vi "2_WF_Anomaly_Detection(Threshold_Evaluation).vi"() -> ()   [LabVIEW 2020]
uses:
  Controls/Optimal_Threshold_Range'.ctl
  <vilib>/Ngene/Deep Learning Toolkit/Toolkit/NN_Network/Controls/NN_Save_Before_Destroy_Options.ctl
  <vilib>/Ngene/Deep Learning Toolkit/Toolkit/NN_Data/subVIs/Get_Data_Vals/2D/NN_Data_Get_ValByRef(2D_SGL).vi
  <vilib>/Ngene/Deep Learning Toolkit/Toolkit/NN_Network/subVIs/NN_Predict/NN_Predict(In1D_Out1D).vi
  <vilib>/Ngene/Deep Learning Toolkit/Toolkit/NN_Data/subVIs/Dataset/NN_Variant_to_DVR/2D/NN_Data_Variant_to_DVR(2D_SGL).vi
  <vilib>/Ngene/Deep Learning Toolkit/Toolkit/Deep_Learning_Toolkit_by_Ngene.lvlib
  <vilib>/Analysis/NI_AALPro.lvlib
panel:
  in  "Validation (Abnormal Samples) dataset path":path=path "D:/working/Anomaly Detection/Validation/Abnormal"
  in  "Validation (Normal Samples) dataset path":path=path "D:/working/Anomaly Detection/Validation/Normal"
  out "Integrals of Normalized Anomaly Score Distributions":cluster{"Axis":dbl[], "Integral X":dbl[]}[](graph)
  out "Anomaly Score Distributions":T1(graph)=[{"X Values"=array[700 elements], "Histogram: h(x)"=[0, 0, 0, 0, 0, 0, 0, 0, 0, 0, 0, 0, 0, 0, 0, 0, 0, 0, 0, 0, 0, 0, 0, 0, 0, 0, 0, 0, 0, 0, 0, 0, 0, 1, 0, 0, 2, 2, 5, 2, 1, 11, 4, 7, 12, 11, 12, 12, 12, 16, 19, 10, 17, 15, 12, 14, 24, 15, 17, 16, 14, 7, 13, 13, 14, 6, 12, 16, 6, 11, 14, 2, 6, 4, 7, 7, 5, 6, 7, 7, 4, 4, 2, 8, 4, 2, 3, 1, 4, 0, 1, 1, 1, 5, 1, 3, 0, 1, 2, 0, 1, 1, 1, 1, 0, 0, 0, 0, 0, 0, 0, 0, 0, 2, 1, 0, 0, 0, 0, 0, 0, 0, 0, 0, 0, 0, 0, 0, 0, 0, 0, 0, 0, 0, 0, 0, 0, 0, 0, 0, 0, 0, 0, 0, 0, 0, 0, 0, 0, 0, 0, 0, 0, 0, 0, 0, 0, 0, 0, 0, 0, 0, 0, 0, 0, 0, 0, 0, 0, 0, 0, 0, 0, 0, 0, 0, 0, 0, 0, 0, 0, 0, 0, 0, 0, 0, 0, 0, 0, 0, 0, 0, 0, 0, 0, 0, 0, 0, 0, 0, 0, 0, 0, 0, 0, 0, 0, 0, 0, 0, 0, 0, 0, 0, 0, 0, 0, 0, 0, 0, 0, 0, 0, 0, 0, 0, 0, 0, 0, 0, 0, 0, 0, 0, 0, 0, 0, 0, 0, 0, 0, 0, 0, 0, 0, 0, 0, 0, 0, 0, 0, 0, 0, 0, 0, 0, 0, 0, 0, 0, 0, 0, 0, 0, 0, 0, 0, 0, 0, 0, 0, 0, 0, 0, 0, 0, 0, 0, 0, 0, 0, 0, 0, 0, 0, 0, 0, 0, 0, 0, 0, 0, 0, 0, 0, 0, 0, 0, 0, 0, 0, 0, 0, 0, 0, 0, 0, 0, 0, 0, 0, 0, 0, 0, 0, 0, 0, 0, 0, 0, 0, 0, 0, 0, 0, 0, 0, 0, 0, 0, 0, 0, 0, 0, 0, 0, 0, 0, 0, 0, 0, 0, 0, 0, 0, 0, 0, 0, 0, 0, 0, 0, 0, 0, 0, 0, 0, 0, 0, 0, 0, 0, 0, 0, 0, 0, 0, 0, 0, 0, 0, 0, 0, 0, 0, 0, 0, 0, 0, 0, 0, 0, 0, 0, 0, 0, 0, 0, 0, 0, 0, 0, 0, 0, 0, 0, 0, 0, 0, 0, 0, 0, 0, 0, 0, 0, 0, 0, 0, 0, 0, 0, 0, 0, 0, 0, 0, 0, 0, 0, 0, 0, 0, 0, 0, 0, 0, 0, 0, 0, 0, 0, 0, 0, 0, 0, 0, 0, 0, 0, 0, 0, 0, 0, 0, 0, 0, 0, 0, 0, 0, 0, 0, 0, 0, 0, 0, 0, 0, 0, 0, 0, 0, 0, 0, 0, 0, 0, 0, 0, 0, 0, 0, 0, 0, 0, 0, 0, 0, 0, 0, 0, 0, 0, 0, 0, 0, 0, 0, 0, 0, 0, 0, 0, 0, 0, 0, 0, 0, 0, 0, 0, 0, 0, 0, 0, 0, 0, 0, 0, 0, 0, 0, 0, 0, 0, 0, 0, 0, 0, 0, 0, 0, 0, 0, 0, 0, 0, 0, 0, 0, 0, 0, 0, 0, 0, 0, 0, 0, 0, 0, 0, 0, 0, 0, 0, 0, 0, 0, 0, 0, 0, 0, 0, 0, 0, 0, 0, 0, 0, 0, 0, 0, 0, 0, 0, 0, 0, 0, 0, 0, 0, 0, 0, 0, 0, 0, 0, 0, 0, 0, 0, 0, 0, 0, 0, 0, 0, 0, 0, 0, 0, 0, 0, 0, 0, 0, 0, 0, 0, 0, 0, 0, 0, 0, 0, 0, 0, 0, 0, 0, 0, 0, 0, 0, 0, 0, 0, 0, 0, 0, 0, 0, 0, 0, 0, 0, 0, 0, 0, 0, 0, 0, 0, 0, 0, 0, 0, 0, 0, 0, 0, 0, 0, 0, 0, 0, 0, 0, 0, 0, 0, 0, 0, 0, 0, 0, 0, 0, 0, 0, 0, 0, 0, 0, 0, 0, 0, 0, 0, 0, 0, 0, 0, 0, 0, 0, 0, 0, 0, 0, 0, 0, 0, 0, 0, 0, 0, 0, 0, 0, 0, 0, 0, 0, 0, 0, 0, 0, 0]}, {"X Values"=array[700 elements], "Histogram: h(x)"=[0, 0, 0, 0, 0, 0, 0, 0, 0, 0, 0, 0, 0, 0, 0, 0, 0, 0, 0, 0, 0, 0, 0, 0, 0, 0, 0, 0, 0, 0, 0, 0, 0, 0, 0, 0, 0, 0, 0, 0, 0, 0, 0, 0, 0, 0, 0, 0, 0, 0, 0, 0, 0, 0, 0, 0, 0, 0, 0, 0, 0, 0, 0, 0, 0, 0, 0, 0, 0, 0, 0, 0, 0, 0, 0, 0, 0, 0, 0, 0, 0, 0, 0, 0, 0, 0, 0, 0, 0, 0, 0, 0, 0, 0, 0, 0, 0, 0, 0, 0, 0, 0, 0, 0, 0, 0, 0, 0, 0, 0, 0, 0, 0, 0, 0, 0, 0, 0, 0, 0, 0, 0, 0, 0, 0, 0, 0, 0, 0, 0, 0, 0, 0, 0, 0, 0, 0, 0, 0, 0, 0, 0, 0, 0, 0, 0, 0, 0, 0, 0, 0, 0, 0, 0, 0, 0, 0, 0, 0, 0, 0, 0, 0, 0, 0, 0, 0, 0, 0, 0, 1, 0, 0, 0, 0, 0, 1, 0, 0, 0, 0, 0, 0, 1, 0, 0, 0, 0, 0, 1, 0, 2, 2, 0, 0, 1, 2, 0, 0, 1, 0, 1, 2, 1, 5, 1, 0, 2, 3, 0, 0, 0, 4, 3, 2, 1, 2, 1, 2, 6, 1, 0, 0, 5, 0, 0, 2, 4, 1, 6, 0, 0, 4, 2, 2, 3, 4, 3, 3, 2, 2, 4, 4, 1, 6, 0, 3, 1, 1, 1, 2, 1, 0, 3, 2, 3, 2, 1, 2, 3, 4, 3, 1, 1, 1, 4, 3, 3, 3, 1, 1, 1, 4, 0, 2, 0, 2, 4, 2, 1, 1, 1, 1, 1, 0, 1, 0, 1, 1, 1, 1, 0, 2, 4, 1, 0, 2, 0, 0, 0, 0, 1, 1, 2, 0, 1, 0, 1, 2, 0, 1, 1, 0, 2, 2, 1, 1, 0, 1, 1, 3, 0, 1, 0, 0, 1, 1, 0, 1, 5, 2, 0, 2, 1, 1, 2, 1, 0, 0, 0, 1, 0, 2, 1, 0, 0, 0, 0, 0, 1, 2, 0, 1, 0, 0, 1, 0, 1, 1, 0, 3, 0, 0, 0, 4, 0, 0, 1, 0, 0, 2, 1, 3, 1, 2, 1, 2, 3, 1, 3, 2, 1, 3, 0, 2, 2, 1, 1, 0, 1, 0, 1, 4, 1, 1, 0, 1, 1, 1, 0, 0, 3, 0, 0, 3, 1, 2, 3, 2, 1, 0, 1, 2, 1, 1, 2, 1, 1, 3, 3, 1, 1, 1, 2, 1, 3, 3, 4, 2, 1, 1, 1, 0, 2, 0, 0, 5, 0, 0, 0, 2, 1, 2, 1, 4, 0, 1, 2, 0, 1, 1, 1, 3, 2, 1, 2, 2, 1, 0, 1, 0, 1, 1, 3, 2, 0, 2, 0, 1, 1, 0, 1, 1, 1, 2, 1, 1, 0, 0, 0, 0, 0, 0, 0, 0, 0, 0, 0, 1, 0, 0, 0, 1, 0, 1, 0, 1, 0, 0, 0, 0, 0, 0, 1, 0, 0, 0, 0, 0, 0, 0, 0, 0, 0, 0, 0, 0, 0, 0, 0, 0, 0, 0, 0, 0, 0, 0, 0, 0, 1, 0, 0, 0, 0, 0, 0, 0, 0, 0, 0, 2, 0, 0, 0, 0, 0, 0, 0, 0, 0, 0, 0, 0, 0, 0, 0, 0, 0, 0, 1, 0, 1, 1, 0, 1, 1, 0, 0, 0, 1, 0, 0, 0, 1, 1, 0, 2, 0, 2, 1, 2, 2, 0, 1, 0, 0, 1, 1, 1, 1, 2, 2, 1, 1, 0, 0, 0, 0, 3, 2, 1, 3, 1, 1, 2, 0, 4, 1, 1, 1, 0, 0, 1, 2, 1, 0, 5, 2, 1, 3, 0, 2, 1, 3, 0, 3, 2, 2, 0, 1, 0, 1, 2, 1, 1, 2, 3, 1, 0, 2, 0, 0, 0, 0, 0, 0, 1, 0, 0, 0, 0, 0, 0, 1, 1, 0, 0, 1, 2, 0, 0, 0, 0, 0, 0, 0, 1, 0, 0, 0, 0, 0, 0, 0, 0, 0, 0, 0, 0, 0, 0, 0, 0, 0, 0, 0, 0, 0, 0, 0, 0, 0, 0, 0, 0, 0, 0, 0, 0, 0]}]
  out "Optimal Threshold Range":T2={"Start"=0.16499999999999998, "Stop"=0.24214285714285716} {"Stop" format="%#_3g"; "Start" format="%#_3g"}
  in  "Weights File Path":path=path "D:/Ngene/GitHub/deepltk_examples/2_Waveform_Processing/24_Waveform_Anomaly_Detection/working/Anomaly_Detection/Anomaly_Detection_weights_25_06_11__13_26_24.bin"
  in  "CFG file path":path=path "D:/Ngene/GitHub/deepltk_examples/2_Waveform_Processing/24_Waveform_Anomaly_Detection/working/Anomaly_Detection/Anomaly_Detection_net_cfg_25_06_11__13_26_24.cfg"
  # "Overview: This VI is designed to calculate the optimal anomaly threshold.\nRequirements: Deep Learning Toolkit for LabVIEW - https://www.ngene.co/deep-learning-toolkit-for-labview\nInstructions:\n1. Provide \"Network Configuration File Path\" and \"Weight File Path\" generated from \"1_WF_Anomaly_Detection(Training).vi\".\n2. Provide Validation (Normal Samples) and Validation (Abnormal Samples) dataset paths.\n3. Run the VI.\n4.Observe the Range of optimal threshold values.\n5. Choose a value from the range of optimal threshold calculated after the VI stops, and use it as a anomaly detetcion threshold in \"3_WF_Anomaly_Detection(Accuracy_Evaluation).vi\" \n6. Open \"3_WF_Anomaly_Detection(Accuracy_Evaluation).vi\"  to deploy the trained network for inference."
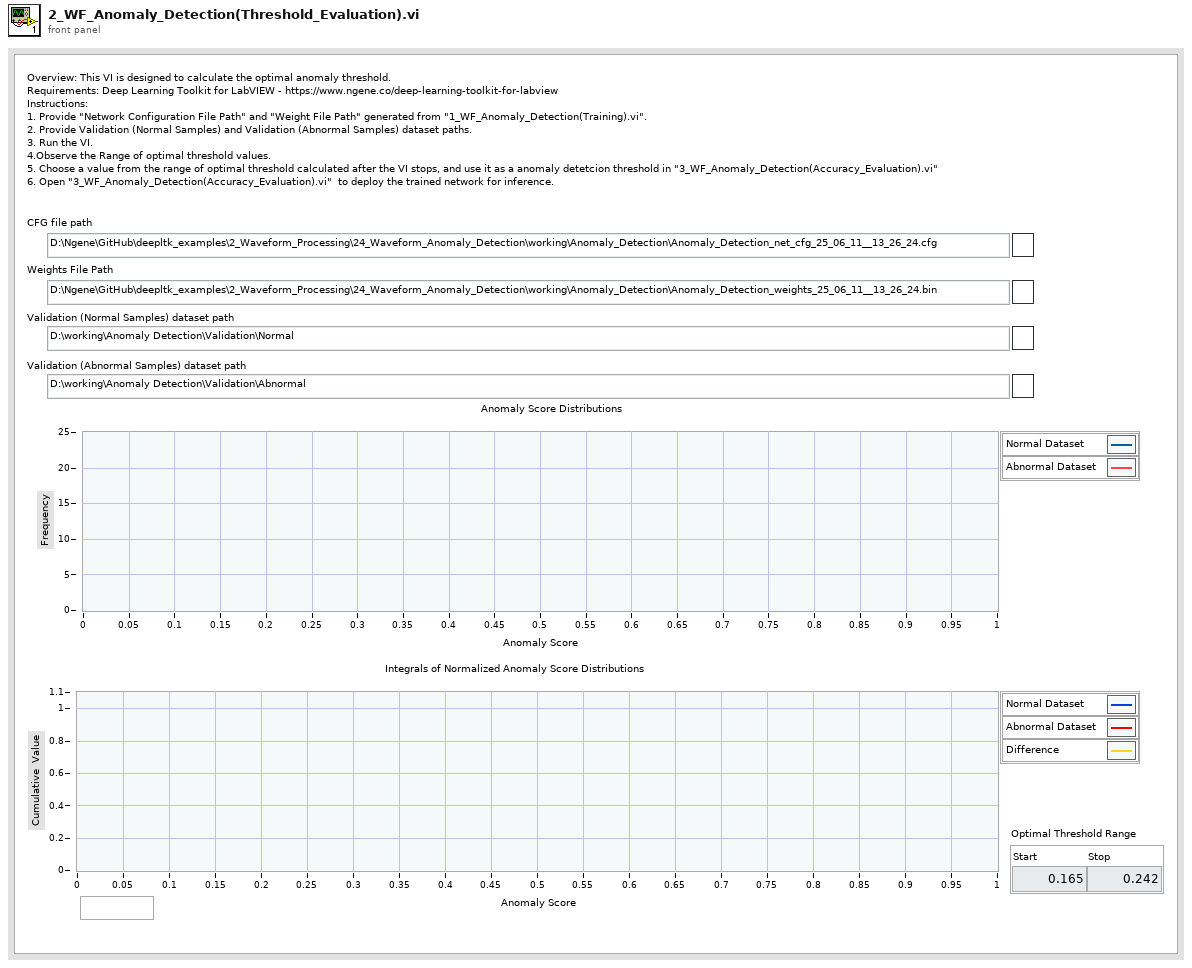
[diagram p1: front panel]
types:
  T1 = cluster{"X Values":dbl[], "Histogram: h(x)":i32[]}[]
  T2 = typedef "Optimal_Threshold_Range'.ctl" = cluster{"Start":dbl, "Stop":dbl}
  T3 = typedef "Deep_Learning_Toolkit_by_Ngene.lvlib/NN_Save_Before_Destroy_Options.ctl" = cluster{"CFG?":bool, "Weights?":bool, "Render?":bool}
  T4 = typedef "Deep_Learning_Toolkit_by_Ngene.lvlib/NN_Config_Params.ctl" = cluster{"Name":string, "mBatch":i32, "NN_Train_Params":T5, "LR_Decay_Policy":T8, "Labels":string[], "Loss":T10, "Max_WS_Size(B)":i64, "DryRun?":bool}
  T5 = typedef "Deep_Learning_Toolkit_by_Ngene.lvlib/NN_Train_Params.ctl" = cluster{"Optimizer":T6, "Beta_1":sgl, "Beta_2":sgl, "Weight Decay(L1)":sgl, "Weight Decay(L2)":sgl, "Data_Sampling":T7}
  T6 = typedef "Deep_Learning_Toolkit_by_Ngene.lvlib/NN_Train_Optimizer.ctl" = enum16{"SGD", "Adam", "Adagrad", "Adadelta", "RMSProp", "Nesterov"}
  T7 = typedef "Deep_Learning_Toolkit_by_Ngene.lvlib/NN_Train_Data_Sampling.ctl" = enum16{"Random", "Sequential"}
  T8 = typedef "Deep_Learning_Toolkit_by_Ngene.lvlib/NN_LR_Policy_Cfg.ctl" = cluster{"Policy_Type":T9, "LR0":dbl, "k":sgl, "WarmUp_Policy":enum16{"Step", "Ramp"}, "WarmUp_Iter":i32, "WarmUp_Ratio":sgl}
  T9 = typedef "Deep_Learning_Toolkit_by_Ngene.lvlib/NN_LR_Policy_Type.ctl" = enum16{"Manual", "Step", "Exp", "1/t"}
  T10 = typedef "Deep_Learning_Toolkit_by_Ngene.lvlib/NN_Loss_Config_Params.ctl" = cluster{"Loss_Type":T11, "Loss_Conf_Params":variant}
  T11 = typedef "Deep_Learning_Toolkit_by_Ngene.lvlib/NN_Loss_Type.ctl" = enum16{"None", "MSE", "CrossEntropy", "YOLO_v2", "YOLO_v4"}
  T12 = typedef "Deep_Learning_Toolkit_by_Ngene.lvlib/NN_Layer_Config_Params.ctl" = cluster{"Layer_Type":T13, "Layer_Conf_Params":variant, "Input Layers":string[]}
  T13 = typedef "Deep_Learning_Toolkit_by_Ngene.lvlib/NN_Layer_Type.ctl" = enum16{"Input1D", "Input3D", "Conv1D", "Conv2D", "Conv2D_Adv", "MaxPool", "AvgPool", "UpSample", "DropOut3D", "ShortCut", "Concat", "SoftMax3D", "FC", "DropOut", "Softmax", "Flatten", "YOLO_v2", "YOLO_v4", "Activation", "BatchNormalization", "LayerNormalization", "Scale", "Unsupported"}
  T14 = typedef "Deep_Learning_Toolkit_by_Ngene.lvlib/NN.ctl" = cluster{"Name":string, "No of Layers":i32, "mBatch":i32, "Layers":T15[], "Dimty":T16, "Dims_In":T17, "Dims_Out":T17, "Working_Dir":path, "Train?":bool, "Train_Params":T5, "LR_Update_Policy":T8, "Session Data":T18, "Ground_truth":T19, "NNg_hdls":T20, "NN_Device":T21, "GPU Id":i32, "Labels":string[], "Loss_Type":T11, "Loss_Cfg_Prms":variant, "NNG_WS":T22, "DryRun?":bool}
  T15 = typedef "Deep_Learning_Toolkit_by_Ngene.lvlib/NN_Layer_ref.ctl" = refnum<file>
  T16 = typedef "Deep_Learning_Toolkit_by_Ngene.lvlib/NN_In_Out_Dim-ty.ctl" = enum8{"In1D_Out1D", "In3D_Out1D", "In3D_Out3D", "In3D_OutBBox"}
  T17 = typedef "Deep_Learning_Toolkit_by_Ngene.lvlib/NN_Dims(C,H,W).ctl" = cluster{"C":i32, "H":i32, "W":i32}
  T18 = typedef "Deep_Learning_Toolkit_by_Ngene.lvlib/NN_Train_Session_Data.ctl" = cluster{"Epochs":sgl, "Tot_Iter":i32, "LR":sgl, "LR_iter":i32}
  T19 = typedef "Deep_Learning_Toolkit_by_Ngene.lvlib/NN_Ground_truth.ctl" = cluster{"Y":variant}
  T20 = typedef "Deep_Learning_Toolkit_by_Ngene.lvlib/nng_cuda_handles.ctl" = cluster{"cudnn":u64, "cublas":u64, "stream":u64, "curand":u64}
  T21 = typedef "Deep_Learning_Toolkit_by_Ngene.lvlib/NN_Device.ctl" = enum16{"CPU", "GPU"}
  T22 = typedef "Deep_Learning_Toolkit_by_Ngene.lvlib/NNG_WS.ctl" = cluster{"NNG_WS_Mem":T23, "Max_WS_Size":i64}
  T23 = typedef "Deep_Learning_Toolkit_by_Ngene.lvlib/NNg_WS_Mem_DVR.ctl" = refnum<data-value>
  T24 = typedef "Deep_Learning_Toolkit_by_Ngene.lvlib/NN_DataSet(In1D_Out1D).ctl" = cluster{"Inputs Ref.":variant, "Outputs Ref.":T25, "Dims_In":i32, "Dataset_Size":i32, "Dims_Out":i32, "Labels":string[], "File Paths":path[], "Custom_Data":variant}
  T25 = typedef "Deep_Learning_Toolkit_by_Ngene.lvlib/NN_Data_ref(2D_SGL).ctl" = refnum<data-value>
  T26 = cluster{"X Values":dbl[], "Histogram: h(x)":i32[]}
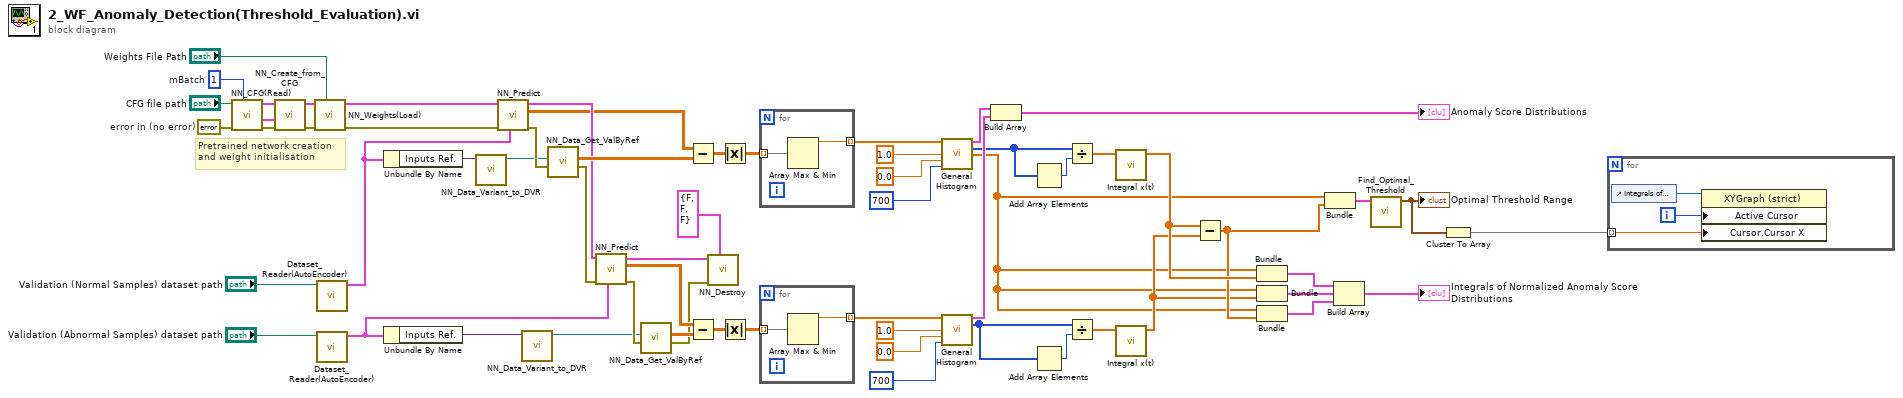
[diagram p0: block diagram]
diagram:
  w56 = 1  # mBatch
  w61 = errorcluster {"status"=FALSE, "code"=0, "source"=""}  # error in (no error)
  # "Pretrained network creation\nand weight initialisation"
  n1 = call <vilib>:"NN_CFG(Read).vi"("mBatch"=w56, "error in (no error)"=w61, "CFG file path"="CFG file path") -> ("error out"=w59:errorcluster, "Net_Cfg"=w60:T4, "Layer_Cfg"=w58:T12[])  [unwired: 6 in]
  n2 = call <vilib>:"NN_Create_from_CFG.vi"("error in (no error)"=w59, "Net_Cfg"=w60, "Layer_Cfg"=w58) -> ("error out"=w62:errorcluster, "NN out"=w57:T14)  [unwired: 7 in]
  n3 = call <vilib>:"NN_Weights(Load).vi"("Weight File Path"="Weights File Path", "error in (no error)"=w62, "NN in"=w57) -> ("error out"=w24:errorcluster, "NN out"=w25:T14)  [unwired: 7 in]
  n4 = call "Dataset_Reader(AutoEncoder).vi"("Train dataset path"="Validation (Normal Samples) dataset path") -> ("Dataset"=w13:T24)  [unwired: 9 in, 1 out]
  n5 = call "Dataset_Reader(AutoEncoder).vi"("Train dataset path"="Validation (Abnormal Samples) dataset path") -> ("Dataset"=w14:T24)  [unwired: 9 in, 1 out]
  n6 = Unbundle By Name(w13) -> ("Inputs Ref."=w12:variant)
  n7 = Unbundle By Name(w14) -> ("Inputs Ref."=w47:variant)
  n8 = call-poly <vilib>:"NN_Data_Variant_to_DVR.vi"("Inputs Ref."=w12) -> ("DVR(2D_SGL)"=w4:T25)  [unwired: 9 in, 1 out]
  n9 = call-poly <vilib>:"NN_Predict.vi"("Dataset"=w13, "error in (no error)"=w24, "NN in"=w25) -> ("error out"=w53:errorcluster, "Predictions"=w43:sgl[][], "NN out"=w49:T14)  [unwired: 6 in]
  n10 = call-poly <vilib>:"NN_Data_Variant_to_DVR.vi"("Inputs Ref."=w47) -> ("DVR(2D_SGL)"=w5:T25)  [unwired: 9 in, 1 out]
  n11 = call-poly <vilib>:"NN_Data_Get_ValByRef.vi"("error in (no error)"=w53, "DVR(2D_SGL)"=w4) -> ("error out"=w50:errorcluster, "Value(2D_SGL)"=w52:sgl[][])  [unwired: 6 in]
  n12 = call-poly <vilib>:"NN_Predict.vi"("Dataset"=w14, "error in (no error)"=w50, "NN in"=w49) -> ("error out"=w46:errorcluster, "Predictions"=w44:sgl[][], "NN out"=w3:T14)  [unwired: 6 in]
  n13 = call-poly <vilib>:"NN_Data_Get_ValByRef.vi"("error in (no error)"=w46, "DVR(2D_SGL)"=w5) -> ("error out"=w2:errorcluster, "Value(2D_SGL)"=w45:sgl[][])  [unwired: 6 in]
  n14 = Subtract(x=w43, y=w52) -> (x-y=w51:sgl[][])
  n15 = Subtract(x=w44, y=w45) -> (x-y=w48:sgl[][])
  n16 = call <vilib>:"NN_Destroy.vi"("Save (T, T, T)"=T3 {"CFG?"=FALSE, "Weights?"=FALSE, "Render?"=FALSE}, "error in (no error)"=w2, "NN in"=w3) -> ()  [unwired: 7 in, 2 out]
  n17 = Absolute Value(x=w51) -> (abs(x)=w42:sgl[][])
  n18 = Absolute Value(x=w48) -> (abs(x)=w41:sgl[][])
  n19 = for {
    tunnel: w42 -> [w64] mode=indexing
    tunnel: [w63] -> w15 mode=indexing
    n20 = Array Max & Min(array=w64) -> (max value=w63:sgl)  [unwired: 3 out]
  }
  n21 = for {
    tunnel: w41 -> [w66] mode=indexing
    tunnel: [w65] -> w16 mode=indexing
    n22 = Array Max & Min(array=w66) -> (max value=w65:sgl)  [unwired: 3 out]
  }
  n23 = call <vilib>:"General Histogram.vi"("X"=w15, "max"=1.0, "min"=0.0, "# bins"=700) -> ("Histogram Graph"=w29:T26, "Histogram"=w27:i32[], "Axis"=w17:dbl[])  [unwired: 7 in, 2 out]
  n24 = call <vilib>:"General Histogram.vi"("X"=w16, "max"=1.0, "min"=0.0, "# bins"=700) -> ("Histogram Graph"=w28:T26, "Histogram"=w32:i32[])  [unwired: 7 in, 3 out]
  n25 = Build Array(w29, w28) -> (→"Anomaly Score Distributions":T1)
  n26 = Add Array Elements(numeric array=w27) -> (sum=w30:i32)
  n27 = Add Array Elements(numeric array=w32) -> (sum=w31:i32)
  n28 = Divide(x=w27, y=w30) -> (x/y=w33:dbl[])
  n29 = Divide(x=w32, y=w31) -> (x/y=w34:dbl[])
  n30 = call <vilib>:"Integral x(t).vi"("X"=w33) -> ("Integral X"=w22:dbl[])  [unwired: 9 in, 1 out]
  n31 = call <vilib>:"Integral x(t).vi"("X"=w34) -> ("Integral X"=w20:dbl[])  [unwired: 9 in, 1 out]
  n32 = Subtract(x=w22, y=w20) -> (x-y=w21:dbl[])
  n33 = Bundle("Axis"=w17, "Integral X"=w22) -> (w8:cluster{"Axis":dbl[], "Integral X":dbl[]})  [unwired: 1 in]
  n34 = Bundle("Axis"=w17, "Integral X"=w20) -> (w9:cluster{"Axis":dbl[], "Integral X":dbl[]})  [unwired: 1 in]
  n35 = Bundle("Axis"=w17, w21) -> (w19:cluster{"Axis":dbl[], dbl[]})  [unwired: 1 in]
  n36 = Bundle("Axis"=w17, w21) -> (w26:cluster{"Axis":dbl[], dbl[]})  [unwired: 1 in]
  n37 = Build Array(w8, w9, w19) -> (→"Integrals of Normalized Anomaly Score Distributions":cluster{"Axis":dbl[], "Integral X":dbl[]}[])
  n38 = call "Find_Optimal_Threshold.vi"("0000000 4"=w26) -> ("Optimal Threshold"=w7:T2)  [unwired: 10 in]
  "Optimal Threshold Range" <- w7
  n39 = Cluster To Array(cluster=w7) -> (array=w6:dbl[])
  n40 = for {
    tunnel: w6 -> [w67] mode=indexing
    i -> [w68]
    n41 = control-ref of="Integrals of Normalized Anomaly Score Distributions"() -> (w69:refnum<vi>)
    n42 = property class="XYGraph (strict)"(reference=w69, "Active Cursor"=w68, "Cursor.Cursor X"=w67) -> ()  [unwired: 1 in, 2 out]
  }
